vi "Day 2.vi"() -> ()   [LabVIEW 2021]
uses:
  <vilib>/Utility/file.llb/Read Delimited Spreadsheet (string).vi
  <vilib>/regexp/Match Regular Expression.xnode
panel:
  out "answer 1":i32
  out "subarray":string[](array[string])
  in  "Input File":enum32{"example input", "input"}(radio)
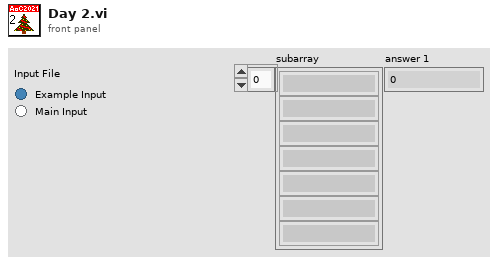
[diagram p1: front panel]
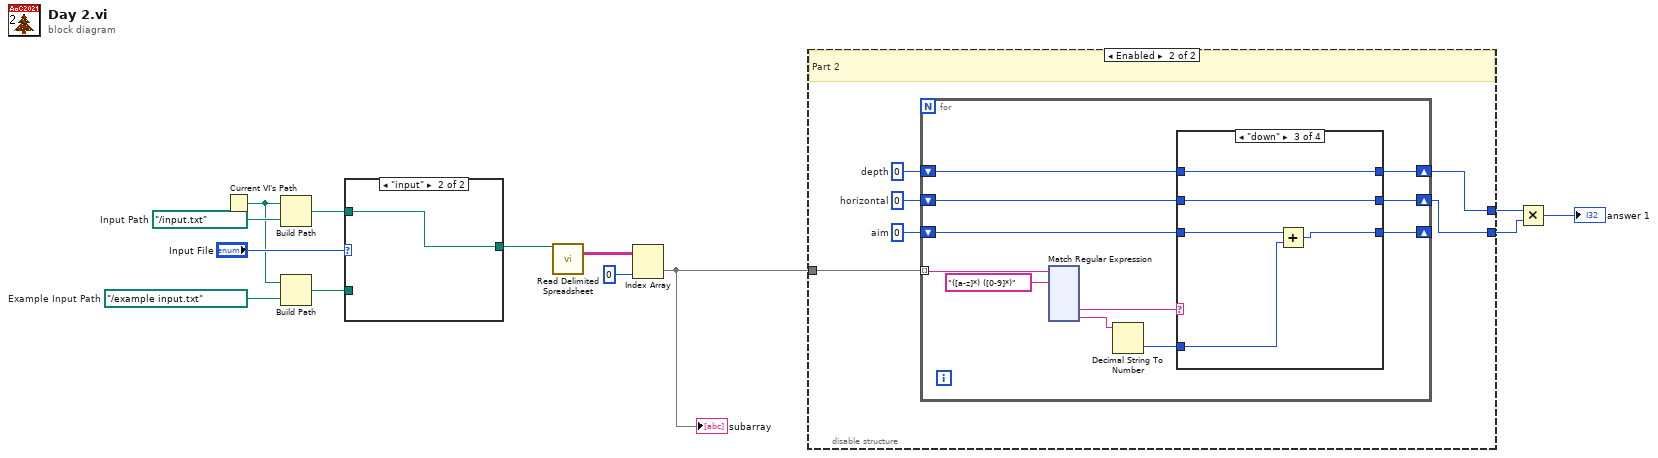
[diagram p0: block diagram]
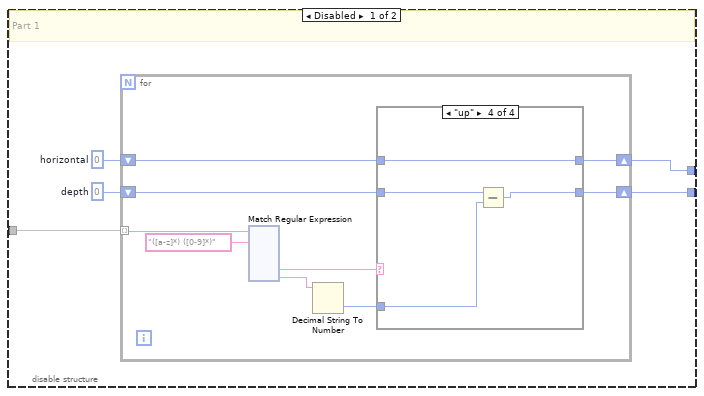
[diagram p2: hidden frame]
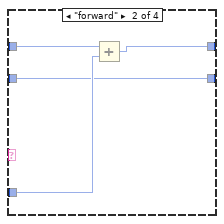
[diagram p4: hidden frame]
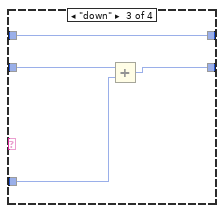
[diagram p5: hidden frame]
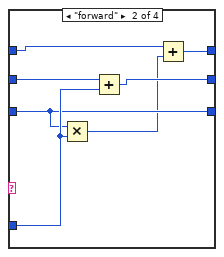
[diagram p7: hidden frame]
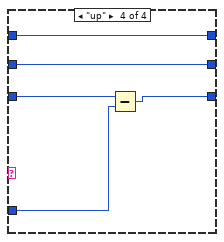
[diagram p8: hidden frame]
diagram:
  w12 = path "../example input.txt"  # Example Input Path
  w13 = path "../input.txt"  # Input Path
  n1 = Current VI's Path() -> (path=w7:path)
  n2 = Build Path(base path=w7, name or relative path=w13) -> (appended path=w10:path)
  n3 = Build Path(base path=w7, name or relative path=w12) -> (appended path=w9:path)
  n4 = case shown="\"input\"" "Input File" {
    tunnel: w10 -> [_ w15]
    tunnel: w9 -> [w14 _]
    tunnel: [w14 w15] -> w8
    frame "example input" {
    }
    frame "input" {
    }
  }
  n5 = call-poly <vilib>:"Read Delimited Spreadsheet.vi"("file path (dialog if empty)"=w8) -> ("all rows"=w6:string[][])  [unwired: 9 in, 5 out]
  n6 = Index Array(array=w6, index (col)=0 ("disabled index (col)")) -> (element=w4:string[])  [unwired: 1 in]
  "subarray" <- w4
  n7 = disable-structure shown="Enabled" {
    disable-tunnel: w4 -> [w20 w169]
    disable-tunnel: [w17 w164] -> w3
    disable-tunnel: [w16 w165] -> w2
    frame Disabled {
      w18 = 0  # depth
      w19 = 0  # horizontal
      # "Part 1"
      n8 = for {
        tunnel: w20 -> [w29] mode=indexing
        shift-right: [w21] -> w17
        shift-left: w19 -> [w26]
        shift-right: [w22] -> w16
        shift-left: w18 -> [w23]
        n9 = xnode "Match Regular Expression"("input string"=w29, "regular expression"="([a-z]*) ([0-9]*)") -> ("submatch 1"=w27:string, "submatch 2"=w25:string)  [unwired: 4 in, 5 out]
        n10 = Decimal String To Number(string=w25) -> (number=w24:i32)  [unwired: 2 in, 1 out]
        n11 = case shown="\"up\"" w27 {
          tunnel: w26 -> [w31 w35 w36 w40]
          tunnel: w24 -> [_ w34 w38 w42]
          tunnel: w23 -> [w30 w33 w39 w43]
          tunnel: [w30 w33 w37 w41] -> w22
          tunnel: [w31 w32 w36 w40] -> w21
          frame Default {
          }
          frame "forward" {
            n12 = Add(x=w35, y=w34) -> (x+y=w32:i32)
          }
          frame "down" {
            n13 = Add(x=w39, y=w38) -> (x+y=w37:i32)
          }
          frame "up" {
            n14 = Subtract(x=w43, y=w42) -> (x-y=w41:i32)
          }
        }
      }
    }
    frame Enabled {
      w166 = 0  # depth
      w167 = 0  # aim
      w168 = 0  # horizontal
      # "Part 2"
      n15 = for {
        tunnel: w169 -> [w180] mode=indexing
        shift-right: [w172] -> w165
        shift-left: w168 -> [w177]
        shift-right: [w173] -> _
        shift-left: w167 -> [w174]
        shift-right: [w170] -> w164
        shift-left: w166 -> [w171]
        n16 = xnode "Match Regular Expression"("input string"=w180, "regular expression"="([a-z]*) ([0-9]*)") -> ("submatch 1"=w178:string, "submatch 2"=w176:string)  [unwired: 4 in, 5 out]
        n17 = Decimal String To Number(string=w176) -> (number=w175:i32)  [unwired: 2 in, 1 out]
        n18 = case shown="\"down\"" w178 {
          tunnel: w177 -> [w183 w190 w192 w197]
          tunnel: w175 -> [_ w188 w194 w199]
          tunnel: w174 -> [w182 w187 w195 w200]
          tunnel: [w182 w187 w193 w198] -> w173
          tunnel: [w183 w189 w192 w197] -> w172
          tunnel: w171 -> [w181 w186 w191 w196]
          tunnel: [w181 w184 w191 w196] -> w170
          frame Default {
          }
          frame "forward" {
            n19 = Multiply(x=w187, y=w188) -> (x*y=w185:i32)
            n20 = Add(x=w190, y=w188) -> (x+y=w189:i32)
            n21 = Add(x=w186, y=w185) -> (x+y=w184:i32)
          }
          frame "down" {
            n22 = Add(x=w195, y=w194) -> (x+y=w193:i32)
          }
          frame "up" {
            n23 = Subtract(x=w200, y=w199) -> (x-y=w198:i32)
          }
        }
      }
    }
  }
  n24 = Multiply(x=w3, y=w2) -> (x*y=→"answer 1":i32)
